vi "FINAL2.vi"() -> ()   [LabVIEW 2022 SP3]
panel:
  in  "dt 2":dbl(slide) scale=0.0..10.0
  in  "Kp2":dbl(knob) scale=0.0..40.0
  in  "Ki2":dbl(knob) scale=0.0..5.0
  in  "Kd2":dbl(knob) scale=0.0..5.0
  out "Theta2_actual":dbl(slide) scale=0.0..100.0
  in  "Theta2_ref":dbl(slide) scale=0.0..40.0
  in  "Theta1_ref":dbl(slide) scale=0.0..40.0
  out "Error Chart":dbl[](graph)
  out "XY RobotArm":cluster{dbl[], dbl[]}(graph)
  out "Error 2":dbl(knob) scale=0.0..10.0
  out "Error 1":dbl(knob) scale=0.0..10.0
  out "Y":dbl(knob) scale=0.0..40.0
  out "X":dbl(knob) scale=0.0..40.0
  out "Theta1_actual":dbl(slide) scale=0.0..100.0
  in  "Reset":bool
  in  "Kd1":dbl(knob) scale=0.0..5.0
  in  "Ki1":dbl(knob) scale=0.0..5.0
  in  "Kp1":dbl(knob) scale=0.0..40.0
  in  "dt":dbl(slide) scale=0.0..10.0
  in  "L2":dbl(slide) scale=0.0..10.0
  in  "L1":dbl(slide) scale=0.0..10.0
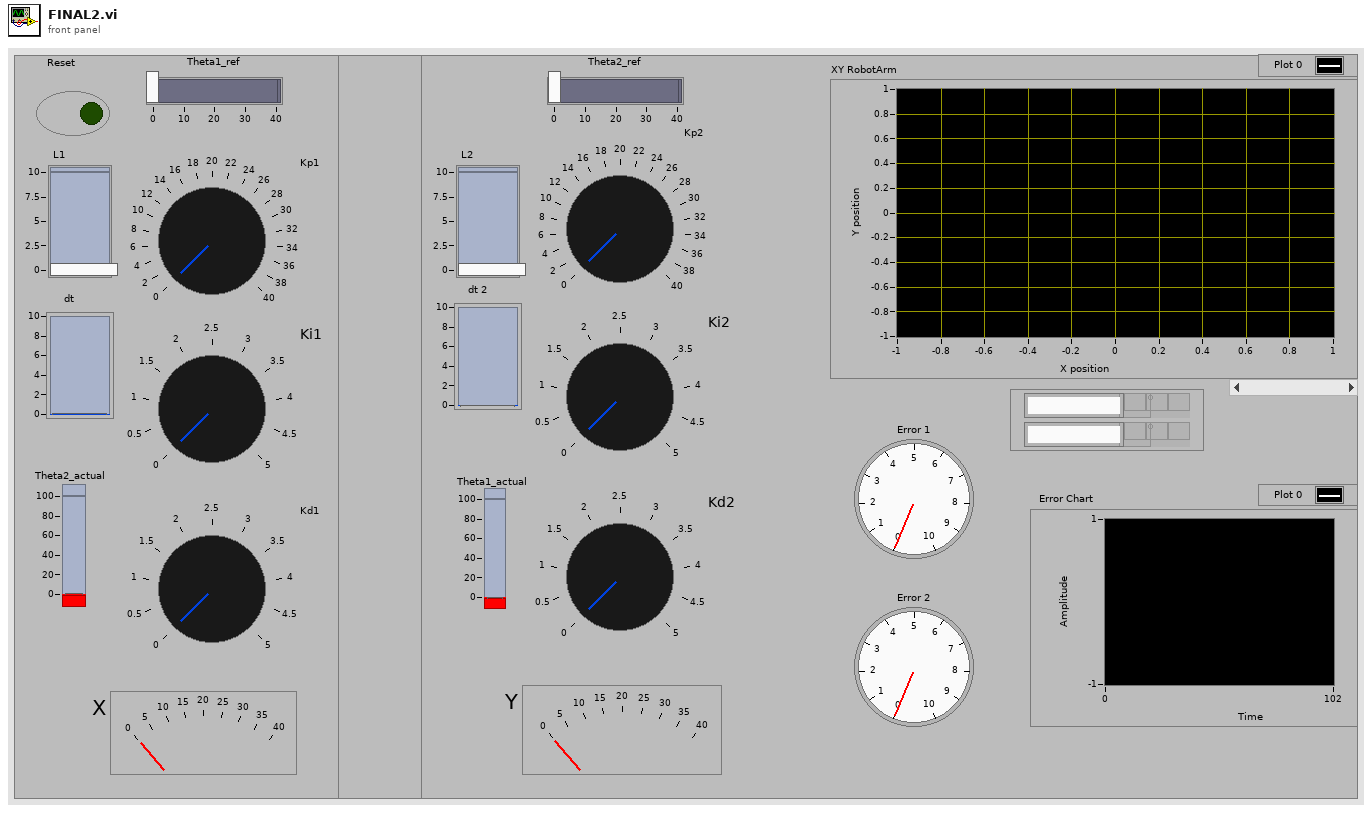
[diagram p1: front panel]
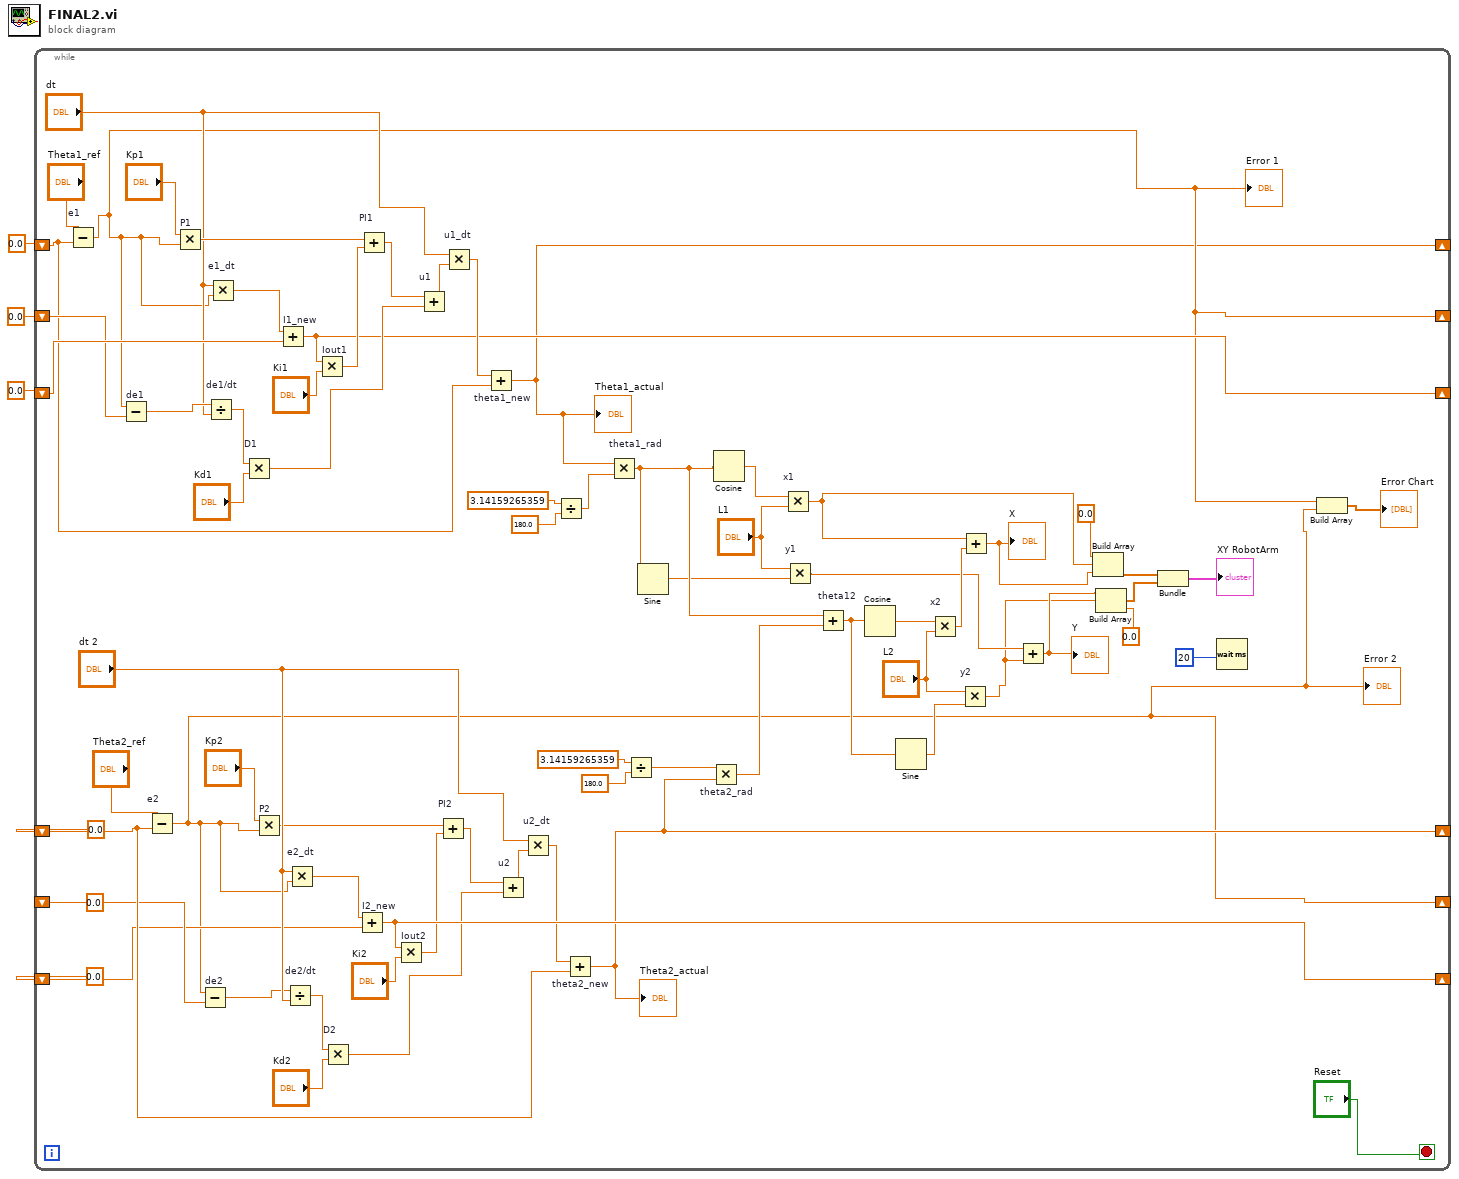
[diagram p0: block diagram]
diagram:
  n1 = while {
    shift-right: [w8] -> _
    shift-left: 0.0 -> [w59]
    shift-right: [w15] -> _
    shift-left: 0.0 -> [w69]
    shift-right: [w57] -> _
    shift-left: 0.0 -> [w72]
    shift-right: [w32] -> _
    shift-left: 0.0 -> [w54]
    shift-right: [w13] -> _
    shift-left: 0.0 -> [w44]
    shift-right: [w56] -> _
    shift-left: 0.0 -> [w41]
    stop <- "Reset" stop-if-true
    n2 = Subtract "e1"(x="Theta1_ref", y=w59) -> (x-y=w15:dbl)
    "Error 1" <- w15
    n3 = Subtract "de1"(x=w15, y=w69) -> (x-y=w68:dbl)
    n4 = Subtract "e2"(x="Theta2_ref", y=w54) -> (x-y=w13:dbl)
    "Error 2" <- w13
    n5 = Multiply "P1"(x="Kp1", y=w15) -> (x*y=w65:dbl)
    n6 = Subtract "de2"(x=w13, y=w44) -> (x-y=w45:dbl)
    n7 = Divide "de1/dt"(x=w68, y="dt") -> (x/y=w67:dbl)
    n8 = Multiply "e1_dt"(x="dt", y=w15) -> (x*y=w71:dbl)
    n9 = Multiply "D1"(x=w67, y="Kd1") -> (x*y=w62:dbl)
    n10 = Multiply "P2"(x="Kp2", y=w13) -> (x*y=w48:dbl)
    n11 = Add "I1_new"(x=w71, y=w72) -> (x+y=w57:dbl)
    n12 = Divide "de2/dt"(x=w45, y="dt 2") -> (x/y=w46:dbl)
    n13 = Multiply "e2_dt"(x="dt 2", y=w13) -> (x*y=w42:dbl)
    n14 = Multiply "Iout1"(x=w57, y="Ki1") -> (x*y=w64:dbl)
    n15 = Multiply "D2"(x=w46, y="Kd2") -> (x*y=w51:dbl)
    n16 = Add "I2_new"(x=w42, y=w41) -> (x+y=w56:dbl)
    n17 = Add "PI1"(x=w65, y=w64) -> (x+y=w63:dbl)
    n18 = Multiply "Iout2"(x=w56, y="Ki2") -> (x*y=w49:dbl)
    n19 = Add "u1"(x=w63, y=w62) -> (x+y=w60:dbl)
    n20 = Add "PI2"(x=w48, y=w49) -> (x+y=w50:dbl)
    n21 = Multiply "u1_dt"(x="dt", y=w60) -> (x*y=w58:dbl)
    n22 = Add "theta1_new"(x=w58, y=w59) -> (x+y=w8:dbl)
    "Theta1_actual" <- w8
    n23 = Add "u2"(x=w50, y=w51) -> (x+y=w53:dbl)
    n24 = Multiply "u2_dt"(x="dt 2", y=w53) -> (x*y=w55:dbl)
    n25 = Divide(x=3.14159265359, y=180.0) -> (x/y=w36:dbl)
    n26 = Add "theta2_new"(x=w55, y=w54) -> (x+y=w32:dbl)
    "Theta2_actual" <- w32
    n27 = Multiply "theta1_rad"(x=w8, y=w36) -> (x*y=w29:dbl)
    n28 = Divide(x=3.14159265359, y=180.0) -> (x/y=w33:dbl)
    n29 = Sine(x=w29) -> (sin(x)=w27:dbl)
    n30 = Multiply "theta2_rad"(x=w33, y=w32) -> (x*y=w31:dbl)
    n31 = Cosine(x=w29) -> (cos(x)=w30:dbl)
    n32 = Multiply "x1"(x=w30, y="L1") -> (x*y=w12:dbl)
    n33 = Multiply "y1"(x="L1", y=w27) -> (x*y=w21:dbl)
    n34 = Add "theta12"(x=w29, y=w31) -> (x+y=w24:dbl)
    n35 = Cosine(x=w24) -> (cos(x)=w26:dbl)
    n36 = Sine(x=w24) -> (sin(x)=w23:dbl)
    n37 = Multiply "x2"(x=w26, y="L2") -> (x*y=w25:dbl)
    n38 = Multiply "y2"(x="L2", y=w23) -> (x*y=w11:dbl)
    n39 = Add(x=w12, y=w25) -> (x+y=w19:dbl)
    "X" <- w19
    n40 = Add(x=w21, y=w11) -> (x+y=w20:dbl)
    "Y" <- w20
    n41 = Build Array(0.0, w12, w19) -> (w18:dbl[])
    n42 = Build Array(w20, w11, 0.0) -> (w17:dbl[])
    n43 = Bundle(w18, w17) -> (→"XY RobotArm":cluster{dbl[], dbl[]})  [unwired: 1 in]
    n44 = Wait (ms)(milliseconds to wait=20) -> ()  [unwired: 1 out]
    n45 = Build Array(w15, w13) -> (→"Error Chart":dbl[])
  }
